vi "Build CE Deploy - Refresh Project.vi"(8 "error in":errorcluster, 10 "Project file":path) -> (0 "error out":errorcluster, 2 "dup Project file":path)   [LabVIEW 2021]
doc: "::: CalcExpress Toolkit :::\nCopyright (c) 2000-2026 Konstantin Shifershteyn. All rights reserved."
panel:
  out "size":i32
  out "Pass #":i32
  # "CalcExpress Toolkit\nCopyright (c) 2000-2026 Konstantin Shifershteyn"
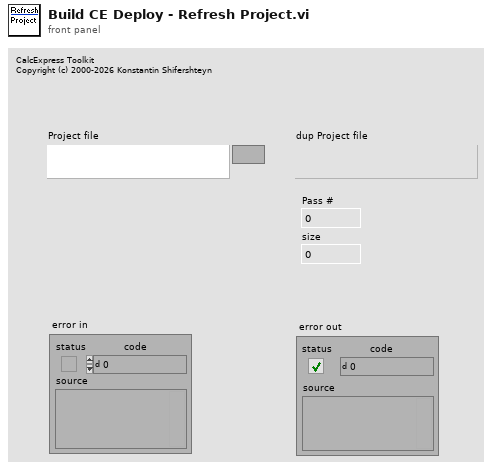
[diagram p1: front panel]
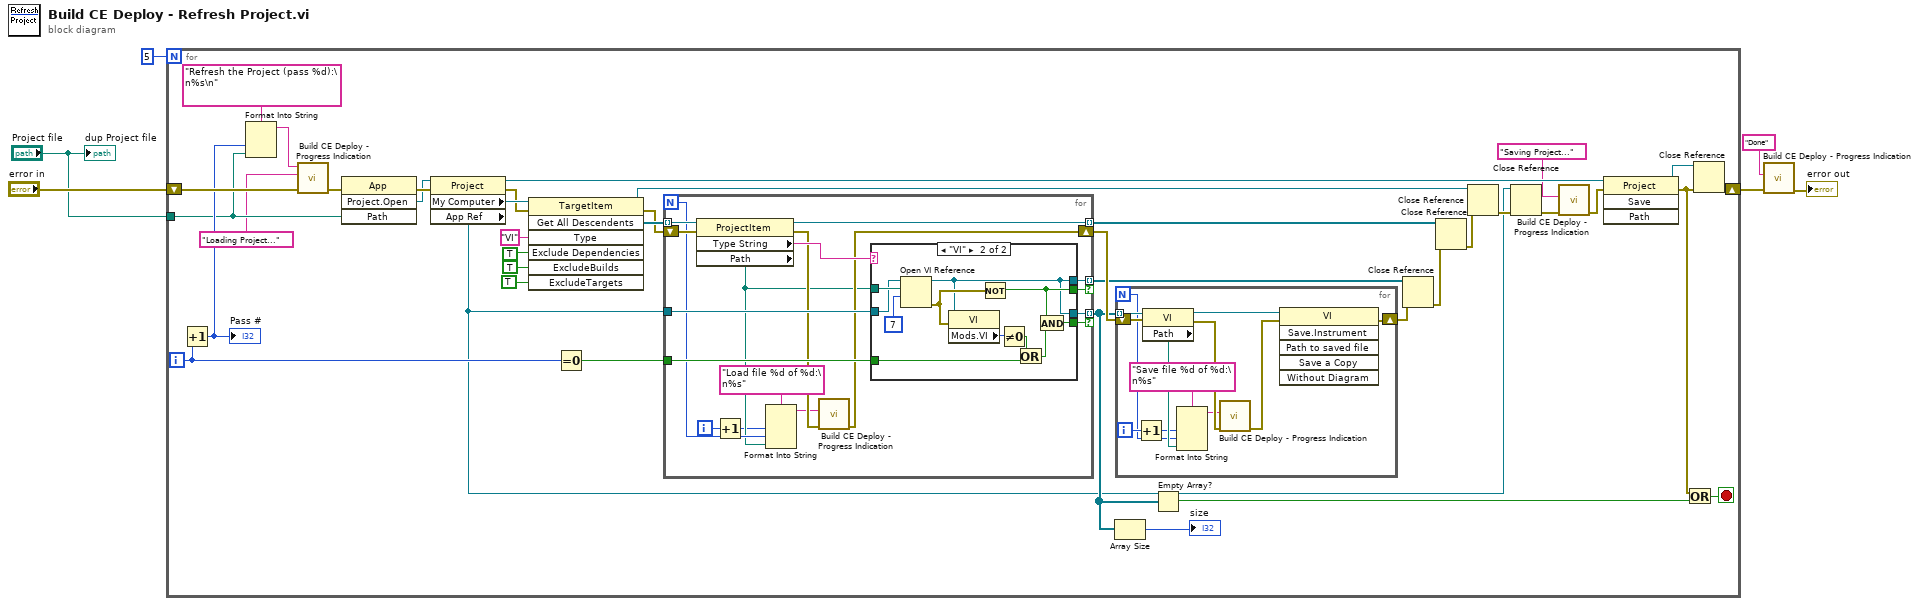
[diagram p0: block diagram]
diagram:
  n1 = for {
    N: 5 -> [_]
    tunnel: "Project file" -> [w8]
    shift-right: [w45] -> w3
    shift-left: "error in" -> [w13]
    i -> [w25]
    stop <- w24 stop-if-true
    n2 = Increment(x=w25) -> (x+1=w9:i32)
    "Pass #" <- w9
    n3 = Format Into String(format string="Refresh the Project (pass %d):\n%s\n", w9, w8) -> (resulting string=w11:string)  [unwired: 2 in, 1 out]
    n4 = call "Build CE Deploy - Progress Indication.vi"("error in"=w13, "message 2"="Loading Project...", "message 1"=w11) -> ("error out"=w12:errorcluster)  [unwired: 8 in]
    n5 = invoke class="App" method="Project.Open"(error in=w12, "Path"=w8) -> (error out=w41:errorcluster, "Project:Open"=w40:refnum<vi>)  [unwired: 2 in, 2 out]
    n6 = property class="Project"(reference=w40, error in=w41) -> (reference out=w26:refnum<vi>, error out=w42:errorcluster, "My Computer"=w43:refnum<vi>, "App Ref"=w17:refnum<vi>)
    n7 = invoke class="TargetItem" method="Get All Descendents"(reference=w43, error in=w42, "Type"="VI", "Exclude Dependencies"=TRUE, "ExcludeBuilds"=TRUE, "ExcludeTargets"=TRUE) -> (reference out=w18:refnum<vi>, error out=w34:errorcluster, "All Descendents"=w35:refnum<vi>[])  [unwired: 1 in, 4 out]
    n8 = Equal To 0?(x=w25) -> (x = 0?=w27:bool)
    n9 = for {
      N -> [w61]
      tunnel: w35 -> [w75] mode=indexing
      shift-right: [w64] -> w33
      shift-left: w34 -> [w74]
      tunnel: w17 -> [w72]
      tunnel: [w71] -> w30 mode=indexing if=w70
      tunnel: [w69] -> w28 mode=indexing if=w68
      tunnel: w27 -> [w67]
      tunnel: [w66] -> w22 mode=indexing
      i -> [w62]
      n10 = property class="ProjectItem"(reference=w75, error in=w74) -> (reference out=w66:refnum<vi>, error out=w65:errorcluster, "Type String"=w73:string, "Path"=w60:path)
      n11 = Increment(x=w62) -> (x+1=w59:i32)
      n12 = Format Into String(format string="Load file %d of %d:\n%s", w59, w61, w60) -> (resulting string=w58:string)  [unwired: 2 in, 1 out]
      n13 = call "Build CE Deploy - Progress Indication.vi"("error in"=w65, "message 2"=w58) -> ("error out"=w64:errorcluster)  [unwired: 9 in]
      n14 = case shown="\"VI\"" w73 {
        tunnel: w60 -> [_ w86]
        tunnel: w72 -> [_ w85]
        tunnel: [_ w80] -> w71
        tunnel: [_ w81] -> w70
        tunnel: [_ w80] -> w69
        tunnel: [_ w79] -> w68
        tunnel: w67 -> [_ w77]
        frame Default {
        }
        frame "VI" {
          n15 = Open VI Reference(application reference (local)=w85, vi path=w86, options=7) -> (vi reference=w80:refnum<vi>, error out=w82:errorcluster)  [unwired: 3 in]
          n16 = property class="VI"(reference=w80, error in=w82) -> ("Mods.VI"=w83:u64)  [unwired: 2 out]
          n17 = Not(x=w82) -> (.not. x?=w81:bool)
          n18 = Not Equal To 0?(x=w83) -> (x != 0?=w78:bool)
          n19 = Or(x=w78, y=w77) -> (x .or. y?=w76:bool)
          n20 = And(x=w81, y=w76) -> (x .and. y?=w79:bool)
        }
      }
    }
    n21 = Array Size(array=w28) -> (size(s)=→"size":i32)
    n22 = for {
      N -> [w47]
      shift-right: [w57] -> w29
      shift-left: w33 -> [w55]
      tunnel: w28 -> [w56] mode=indexing
      i -> [w48]
      n23 = Increment(x=w48) -> (x+1=w46:i32)
      n24 = property class="VI"(reference=w56, error in=w55) -> (reference out=w54:refnum<vi>, error out=w53:errorcluster, "Path"=w49:path)
      n25 = Format Into String(format string="Save file %d of %d:\n%s", w46, w47, w49) -> (resulting string=w51:string)  [unwired: 2 in, 1 out]
      n26 = call "Build CE Deploy - Progress Indication.vi"("error in"=w53, "message 2"=w51) -> ("error out"=w52:errorcluster)  [unwired: 9 in]
      n27 = invoke class="VI" method="Save.Instrument"(reference=w54, error in=w52) -> (error out=w57:errorcluster)  [unwired: 4 in, 5 out]
    }
    n28 = Empty Array?(array=w28) -> (empty?=w32:bool)
    n29 = Close Reference(reference=w30, error in (no error)=w29) -> (error out=w21:errorcluster)
    n30 = Close Reference(reference=w22, error in (no error)=w21) -> (error out=w20:errorcluster)
    n31 = Close Reference(reference=w18, error in (no error)=w20) -> (error out=w19:errorcluster)
    n32 = Close Reference(reference=w17, error in (no error)=w19) -> (error out=w16:errorcluster)
    n33 = call "Build CE Deploy - Progress Indication.vi"("error in"=w16, "message 2"="Saving Project...") -> ("error out"=w14:errorcluster)  [unwired: 9 in]
    n34 = invoke class="Project" method="Save"(reference=w26, error in=w14) -> (reference out=w44:refnum<vi>, error out=w23:errorcluster)  [unwired: 2 in, 2 out]
    n35 = Or(x=w23, y=w32) -> (x .or. y?=w24:bool)
    n36 = Close Reference(reference=w44, error in (no error)=w23) -> (error out=w45:errorcluster)
  }
  n37 = call "Build CE Deploy - Progress Indication.vi"("error in"=w3, "message 2"="Done") -> ("error out"=→"error out":errorcluster)  [unwired: 9 in]
  "dup Project file" <- "Project file"
